vi "onStop.vi"(8 "error in (no error)":errorcluster, 11 "Client in":refnum<class "Client.lvclass">) -> (0 "error out":errorcluster, 3 "Client out":refnum<class "Client.lvclass">)   [LabVIEW 2013, in "MQTT Client.lvlib" / "Client.lvclass"]
uses:
  Client.lvclass
  <vilib>/LabVIEW Open Source Project/MQTT Connection/MQTT_Base/Base Class/MQTT_Base.lvclass
  Session.Client/Session.Client.lvclass
  <vilib>/LabVIEW Open Source Project/MQTT Connection/MQTT_Base/Session/Session.lvclass
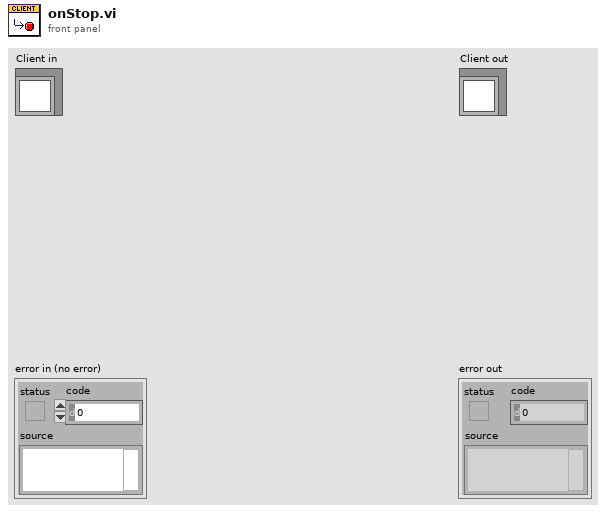
[diagram p1: front panel]
types:
  T1 = typedef "MQTT Client.lvlib/Client.lvclass/Public Events -- cluster.ctl" = cluster{"Connection Status":refnum<user-event>, "Connected":refnum<user-event>, "Application Message":refnum<user-event>}
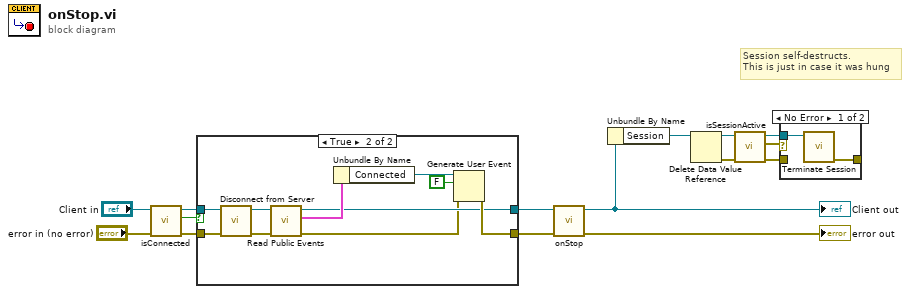
[diagram p0: block diagram]
diagram:
  # "Session self-destructs.\nThis is just in case it was hung"
  n1 = call "isConnected.vi"("error in (no error)"="error in (no error)", "Client in"="Client in") -> ("error out"=w10:errorcluster, "connected"=w8:bool, "Client out"=w9:refnum<class "Client.lvclass">)  [unwired: 7 in]
  n2 = case shown="True" w8 {
    tunnel: [w15 w25] -> w13
    tunnel: [w16 w21] -> w12
    tunnel: w10 -> [w15 w18]
    tunnel: w9 -> [w16 w17]
    frame False {
    }
    frame True {
      n3 = call "Disconnect from Server.vi"("error in (no error)"=w18, "Client in"=w17) -> ("error out"=w20:errorcluster, "Client out"=w22:refnum<class "Client.lvclass">)  [unwired: 7 in, 1 out]
      n4 = call "Read Public Events.vi"("error in (no error)"=w20, "Client in"=w22) -> ("error out"=w19:errorcluster, "Client Public Events"=w23:T1, "Client out"=w21:refnum<class "Client.lvclass">)  [unwired: 7 in]
      n5 = Unbundle By Name(w23) -> ("Connected"=w26:refnum<user-event>)
      n6 = Generate User Event(user event=w26, event data cluster=FALSE ("event data"), error in=w19) -> (error out=w25:errorcluster)  [unwired: 1 in, 1 out]
    }
  }
  n7 = call-parent "onStop.vi"("error in (no error)"=w13, "MQTT_Base in"=w12) -> ("error out"=→"error out":errorcluster, "MQTT_Base out"=w6:refnum<class "Client.lvclass">)  [unwired: 8 in]
  "Client out" <- w6
  n8 = Unbundle By Name(w6) -> ("Session"=w5:refnum<data-value>)
  n9 = Delete Data Value Reference(data value reference=w5) -> (data value=w3:refnum<class "Session.Client.lvclass">, error out=w1:errorcluster)  [unwired: 1 in]
  n10 = call <vilib>:"isSessionActive.vi"("Session in"=w3) -> ("error out"=w2:errorcluster, "Session out"=w4:refnum<class "Session.Client.lvclass">)  [unwired: 9 in]
  n11 = case shown="No Error" w2 {
    tunnel: [w28 _] -> _
    tunnel: w4 -> [w27 _]
    tunnel: w1 -> [_ _]
    frame No Error {
      n12 = call <vilib>:"Terminate Session.vi"("Session in"=w27) -> ("error out"=w28:errorcluster)  [unwired: 8 in, 2 out]
    }
    frame Error {
    }
  }
